vi "Mass Compile VI Helpeks.vi"() -> ()   [LabVIEW 2014]
doc: "::: VI Helpeks :::\nCopyright (c) 2000-2026 Konstantin Shifershteyn. All rights reserved."
uses:
  <vilib>/event_ctls.llb/eventvkey.ctl
  <vilib>/Platform/browser.llb/Open URL in Default Browser (path).vi
panel:
  in  "Cache VIs":u32=50
  in  "<Examples>":bool=TRUE caption="VI Helpeks VIs in <Examples>"
  in  "<Project>":bool=TRUE caption="VI Helpeks VIs in <Project>"
  in  "<vi.lib>":bool=TRUE caption="VI Helpeks VIs in <vi.lib>"
  in  "Open Logfile":bool
  in  "Compile":bool
  in  "Exit":bool
  in  "Log mode":T1(ring)
  in  "Log file":path
  # "Compile parameters"
  # "Compiling log file"
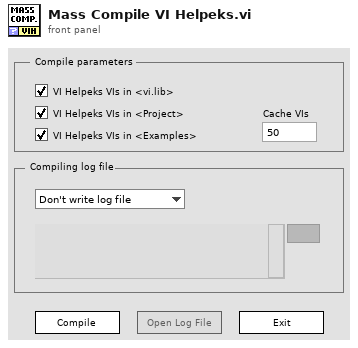
[diagram p1: front panel]
types:
  T1 = enum16{"Don't write log file", "Write new log file", "Append to log file"}
  T2 = typedef "eventvkey.ctl" = enum16{"ASCII", "Enter", "Return", "Shift", "Ctrl", "Alt", "Cmd", "Opt", "Caps", "NumLock", "Clear", "Break", "Up", "Down", "Left", "Right", "Insert", "Delete", "Home", "End", "PageUp", "PageDown", "Escape", "Help", "Pause", "ScrollLock", "F1", "F2", "F3", "F4", "F5", "F6", "F7", "F8", "F9", "F10", "F11", "F12", "F13", "F14", "F15", "F16", "F17", "F18", "F19", "F20", "F21", "F22", "F23", "F24", "Play", "VolumeUp", "VolumeDown", "Mute", "Two Byte Char"}
  T3 = enum8{"Enabled", "Disabled", "Disabled and Grayed Out"}
  T4 = cluster{"Shift":bool, "Ctrl":bool, "Alt":bool, "Cmd":bool, "Opt":bool}
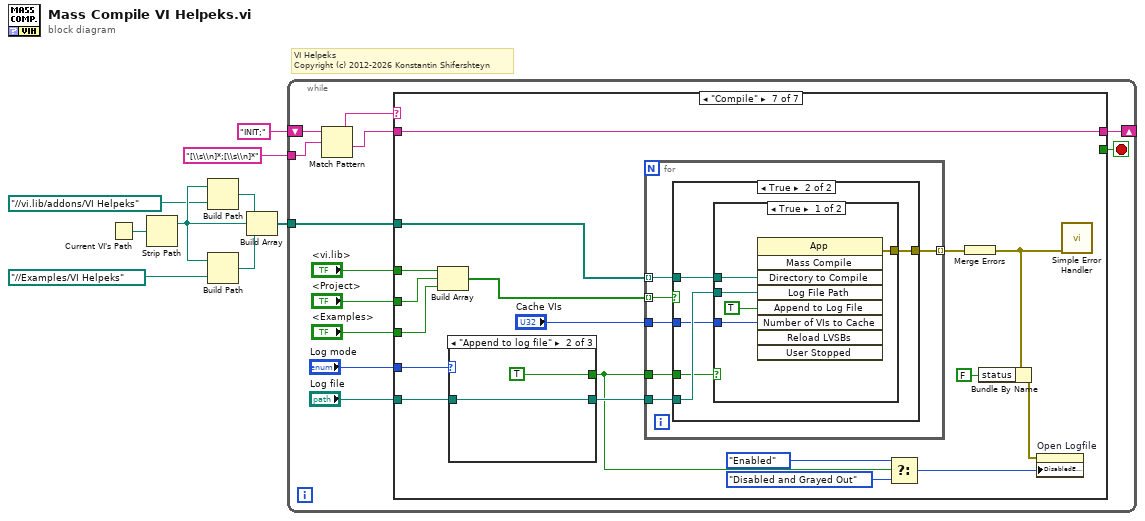
[diagram p0: block diagram]
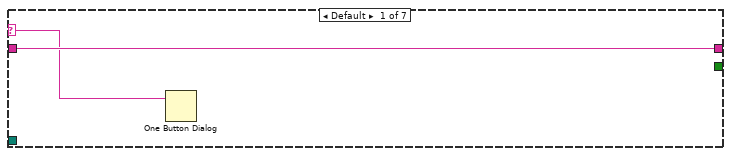
[diagram p2: hidden frame]
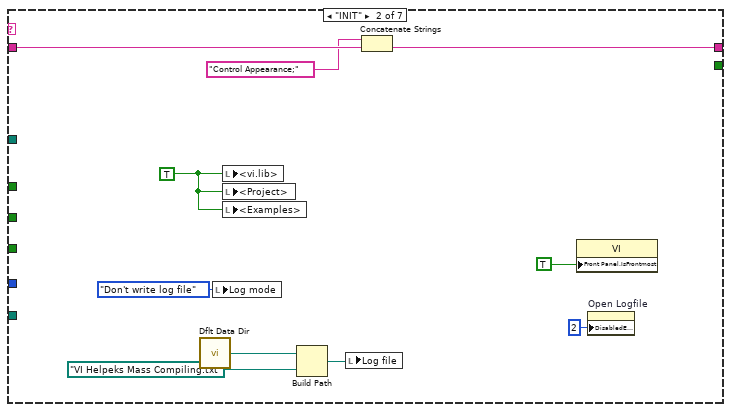
[diagram p3: hidden frame]
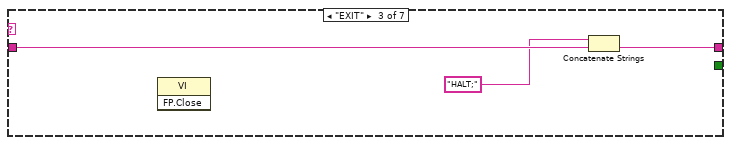
[diagram p4: hidden frame]
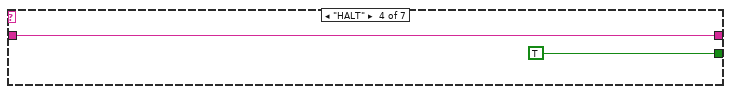
[diagram p5: hidden frame]
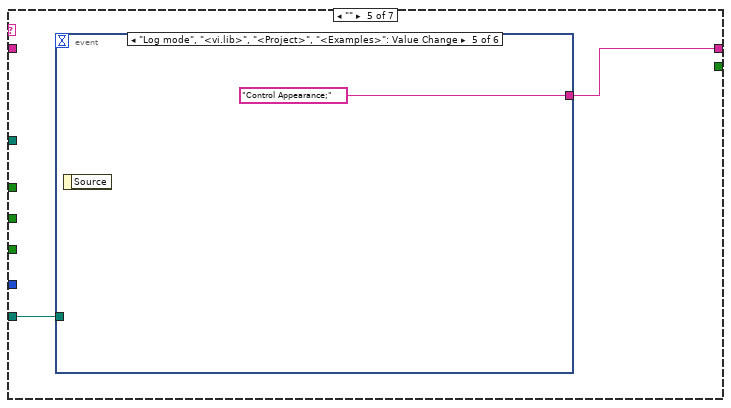
[diagram p6: hidden frame]
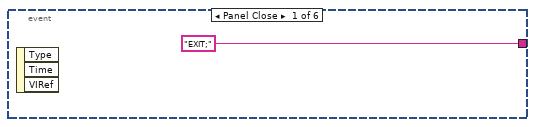
[diagram p7: hidden frame]
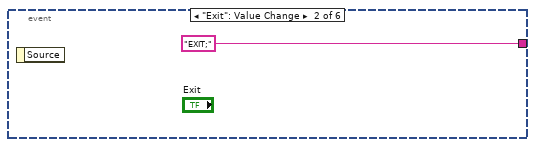
[diagram p8: hidden frame]
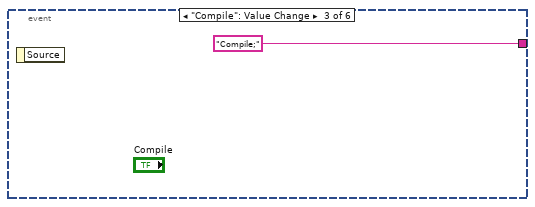
[diagram p9: hidden frame]
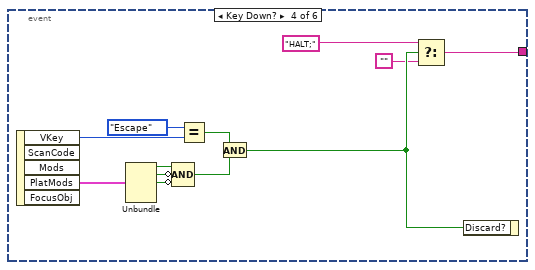
[diagram p10: hidden frame]
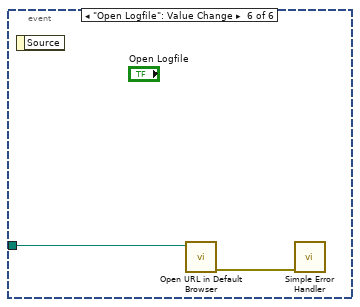
[diagram p11: hidden frame]
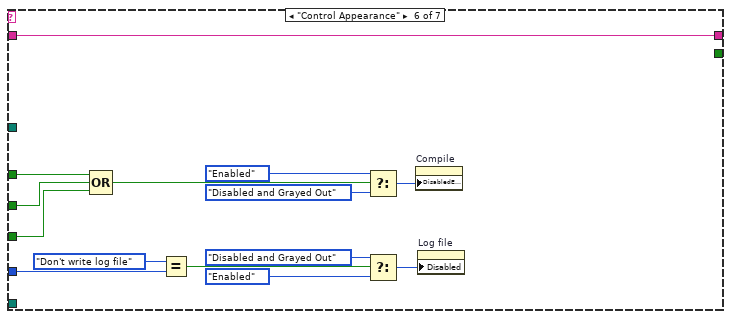
[diagram p12: hidden frame]
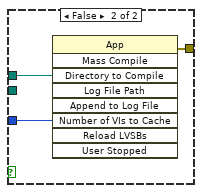
[diagram p14: hidden frame]
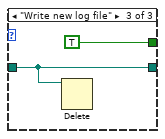
[diagram p16: hidden frame]
diagram:
  # "VI Helpeks\nCopyright (c) 2012-2026 Konstantin Shifershteyn"
  n1 = Current VI's Path() -> (path=w7:path)
  n2 = Strip Path(path=w7) -> (stripped path=w6:path)  [unwired: 1 out]
  n3 = Build Path(base path=w6, name or relative path=path "../../vi.lib/addons/VI Helpeks") -> (appended path=w2:path)
  n4 = Build Path(base path=w6, name or relative path=path "../../Examples/VI Helpeks") -> (appended path=w1:path)
  n5 = Build Array(w2, w6, w1) -> (w3:path[])
  n6 = while {
    shift-right: [w21] -> _
    shift-left: "INIT;" -> [w17]
    tunnel: "[\\s\\n]*;[\\s\\n]*" ("regular expression") -> [w16]
    tunnel: w3 -> [w13]
    stop <- w20 stop-if-true
    n7 = Match Pattern(string=w17, regular expression=w16) -> (before substring=w14:string, after substring=w15:string)  [unwired: 3 out]
    n8 = case shown="\"Compile\"" w14 {
      selector: w14 -> [w22 _ _ _ _ _ _]
      tunnel: w15 -> [w23 w31 w36 w38 _ w72 w90]
      tunnel: [w23 w30 w35 w38 w40 w72 w90] -> w21
      tunnel: [_ _ _ TRUE _ _ _] -> w20
      tunnel: "Log mode" -> [_ _ _ _ _ w71 w89]
      tunnel: "Log file" -> [_ _ _ _ w39 _ w88]
      tunnel: w13 -> [_ _ _ _ _ _ w73]
      tunnel: "<vi.lib>" -> [_ _ _ _ _ w65 w77]
      tunnel: "<Project>" -> [_ _ _ _ _ w64 w76]
      tunnel: "<Examples>" -> [_ _ _ _ _ w63 w75]
      frame Default {
        n9 = One Button Dialog(message=w22) -> ()  [unwired: 1 in, 1 out]
      }
      frame "INIT" {
        w24 = TRUE
        n10 = call <vilib>:"Dflt Data Dir.vi"() -> ("App:Default Data Directory"=w26:path)
        n11 = local write "Log mode"(T1."Don't write log file" ("Log mode")) -> ()
        n12 = local write "<vi.lib>"(w24) -> ()
        n13 = local write "<Project>"(w24) -> ()
        n14 = local write "<Examples>"(w24) -> ()
        n15 = Build Path(base path=w26, name or relative path=path "VI Helpeks Mass Compiling.txt") -> (appended path=w33:path)
        n16 = local write "Log file"(w33) -> ()
        n17 = Concatenate Strings("Control Appearance;", w31) -> (w30:string)
        n18 = property class="VI"("Front Panel.IsFrontmost"=TRUE) -> ()  [unwired: 2 in, 2 out]
        n19 = property on="Open Logfile" class="Bool"("DisabledEnum"=u8 2 ("Control Disable if False")) -> ()  [unwired: 2 in, 2 out]
      }
      frame "EXIT" {
        n20 = invoke class="VI" method="FP.Close"() -> ()  [unwired: 3 in, 3 out]
        n21 = Concatenate Strings("HALT;" ("string"), w36) -> (w35:string)
      }
      frame "HALT" {
      }
      frame "" {
        n22 = event shown="[4] \"Log mode\", \"<vi.lib>\", \"<Project>\", \"<Examples>\": Value Change" {
          selector: _ -> [_ _ _ _ _ _]
          dyn-events: _ -> [_ _ _ _ _ _]
          timeout: _ -> [_ _ _ _ _ _]
          tunnel: ["EXIT;" "EXIT;" "Compile;" w46 "Control Appearance;" _] -> w40
          tunnel: w39 -> [_ _ _ _ _ w58]
          event Panel Close {
            n23 = event-data() -> ()  [unwired: 1 in, 3 out]
          }
          event "Exit": Value Change {
            n24 = event-data() -> ()  [unwired: 1 in, 1 out]
          }
          event "Compile": Value Change {
            n25 = event-data() -> ()  [unwired: 1 in, 1 out]
          }
          event Key Down? {
            n26 = event-data() -> ("VKey"=w54:T2, "PlatMods"=w55:T4)  [unwired: 1 in, 3 out]
            n27 = Unbundle(w55) -> ("Shift"=w52:bool, "Ctrl"=w51:bool, "Alt"=w50:bool)  [unwired: 2 out]
            n28 = Compound Arithmetic op=AND(w52, invert w51, invert w50) -> (w49:bool)
            n29 = Equal?(x=eventvkey."Escape", y=w54) -> (x = y?=w48:bool)
            n30 = And(x=w48, y=w49) -> (x .and. y?=w47:bool)
            n31 = Select(t="HALT;", s=w47, f="") -> (s? t:f=w46:string)
            n32 = event-data("Discard?"=w47) -> ()  [unwired: 1 in, 1 out]
          }
          event "Log mode", "<vi.lib>", "<Project>", "<Examples>": Value Change {
            n33 = event-data() -> ()  [unwired: 1 in, 1 out]
          }
          event "Open Logfile": Value Change {
            n34 = event-data() -> ()  [unwired: 1 in, 1 out]
            n35 = call-poly <vilib>:"Open URL in Default Browser.vi"("path"=w58) -> ("error out"=w57:errorcluster)  [unwired: 5 in, 1 out]
            n36 = call <vilib>:"Simple Error Handler.vi"("error in (no error)"=w57) -> ()  [unwired: 4 in, 5 out]
          }
        }
      }
      frame "Control Appearance" {
        n37 = Compound Arithmetic op=OR(w65, w64, w63) -> (w60:bool)
        n38 = Equal?(x=T1."Don't write log file", y=w71) -> (x = y?=w69:bool)
        n39 = Select(t=T3."Enabled", s=w60, f=T3."Disabled and Grayed Out" ("Disabled")) -> (s? t:f=w59:T3)
        n40 = Select(t=T3."Disabled and Grayed Out", s=w69, f=T3."Enabled" ("Disabled")) -> (s? t:f=w66:T3)
        n41 = property on="Compile" class="Bool"("DisabledEnum"=w59) -> ()  [unwired: 2 in, 2 out]
        n42 = property on="Log file" class="Path"("Disabled"=w66) -> ()  [unwired: 2 in, 2 out]
      }
      frame "Compile" {
        n43 = Build Array(w77, w76, w75) -> (w74:bool[])
        n44 = case shown="\"Append to log file\"" w89 {
          tunnel: w88 -> [_ w111 w113]
          tunnel: [_ w111 w113] -> w87
          tunnel: [_ TRUE TRUE] -> w81
          frame "Don't write log file" {
          }
          frame "Append to log file" {
          }
          frame "Write new log file" {
            n45 = Delete(path (use dialog)=w113) -> ()  [unwired: 4 in, 3 out]
          }
        }
        n46 = for {
          tunnel: w87 -> [w96]
          tunnel: [w95] -> w84 mode=indexing
          tunnel: w81 -> [w94]
          tunnel: "Cache VIs" -> [w93]
          tunnel: w73 -> [w92] mode=indexing
          tunnel: w74 -> [w91] mode=indexing
          n47 = case shown="True" w91 {
            tunnel: w96 -> [_ w101]
            tunnel: [_ w100] -> w95
            tunnel: w94 -> [_ w99]
            tunnel: w92 -> [_ w98]
            tunnel: w93 -> [_ w97]
            frame False {
            }
            frame True {
              n48 = case shown="True" w99 {
                tunnel: w98 -> [w106 w109]
                tunnel: w101 -> [w105 _]
                tunnel: [w103 w108] -> w100
                tunnel: w97 -> [w102 w107]
                frame True {
                  n49 = invoke class="App" method="Mass Compile"("Directory to Compile"=w106, "Log File Path"=w105, "Append to Log File"=TRUE, "Number of VIs to Cache"=w102) -> (error out=w103:errorcluster)  [unwired: 5 in, 8 out]
                }
                frame False {
                  n50 = invoke class="App" method="Mass Compile"("Directory to Compile"=w109, "Number of VIs to Cache"=w107) -> (error out=w108:errorcluster)  [unwired: 7 in, 8 out]
                }
              }
            }
          }
        }
        n51 = Select(t=T3."Enabled", s=w81, f=T3."Disabled and Grayed Out" ("Disabled")) -> (s? t:f=w80:T3)
        n52 = Merge Errors(w84) -> (w78:errorcluster)
        n53 = Bundle By Name(cluster=w78, "status"=FALSE) -> (w86:errorcluster)
        n54 = property on="Open Logfile" class="Bool"(error in=w86, "DisabledEnum"=w80) -> ()  [unwired: 1 in, 2 out]
        n55 = call <vilib>:"Simple Error Handler.vi"("error in (no error)"=w78) -> ()  [unwired: 4 in, 5 out]
      }
    }
  }
